vi "TxBegin_Core.vi"(8 "error in (no error)":errorcluster, 11 "DBC in":refnum<class "DBC.lvclass">) -> (0 "error out":errorcluster, 3 "DBC out":refnum<class "DBC.lvclass">)   [LabVIEW 2020, in "ORM_sqlite_jdp.lvlib" / "DBC.lvclass"]
uses:
  DBC.lvclass
  DBC.lvclass/DBC.ctl
  <vilib>/drjdpowell/SQLite Library/Transaction Helpers/Transaction.lvlib
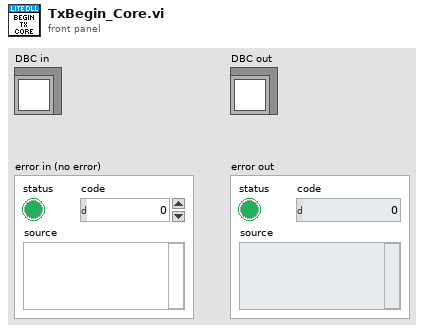
[diagram p1: front panel]
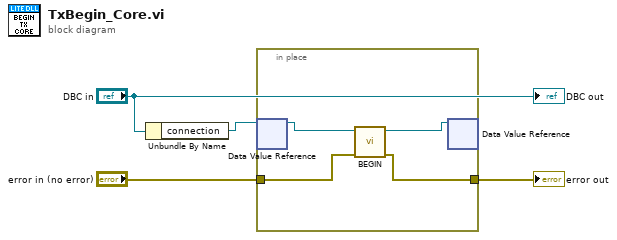
[diagram p0: block diagram]
diagram:
  n1 = Unbundle By Name("DBC in") -> ("connection"=w1:refnum<data-value>)
  n2 = in-place {
    in-place-border: "error in (no error)" -> [w8]
    in-place-border: [w7] -> w2
    n3 = in-place-dvr #1(w1) -> (w6:refnum<class "Connection.lvclass">)  [unwired: 1 out]
    n4 = call <vilib>:"BEGIN.vi"("error in (no error)"=w8, "SQLite Connection in"=w6) -> ("error out"=w7:errorcluster, "SQLite Connection"=w5:refnum<class "Connection.lvclass">)  [unwired: 8 in]
    n5 = in-place-dvr #1(w5) -> ()  [unwired: 2 out]
  }
  "error out" <- w2
  "DBC out" <- "DBC in"
